vi "Define Test Suite (SimpleText Report).vi"(4 "timeout":i32=2000, 5 "register caller level (0)":i32, 6 "Verbose (F)":bool, 8 "error in (no error)":errorcluster, 9 "Report Path":path, 10 "Interactive":bool, 11 "Label (VI Title)":string) -> (0 "error out":errorcluster, 2 "Properties.Suite":refnum<class "Properties.Suite.lvclass">, 3 "Test Suite":refnum<class "Test Suite.lvclass">)   [LabVIEW 2020, in "Caraya.lvlib" / "Test Suite.lvclass"]
doc: "Registers the calling VI as a test suite. If Interactive is True, the interactive user interface is opened when the test suite is executed. If the Report Path is set, a report file will be generated with the test results.\n\n--\nCopyright © 2015 JKI All rights reserved.\n\nAuthor: Tomi Maila <tomi.maila@jki.net>\n\nThis library is provided \"AS IS\" ,WITHOUT WARRANTIES OR\nCONDITIONS OF ANY KIND, either express or implied.\n\nJKI -- jki.net"
uses:
  Test Suite.lvclass
  Properties.Suite/Properties.Suite.lvclass
  C:/projects/caraya/src/classes/Properties/Properties.lvclass
  Test Assert Factory/Test Assert Factory.lvclass
  Test Report.Default/Test Report.Default.lvclass
  C:/projects/caraya/src/classes/Test Report/Test Report.lvclass
  Test Suite.lvclass/Test Suite.ctl
  Properties.Suite/Properties.Suite.lvclass/Properties.Suite.ctl
  Caraya.lvlib
  Assert Factory Manager/Assert Factory Manager.lvclass
  Basic Test Manager/Basic Test Manager.lvclass
  Properties/Properties.lvclass
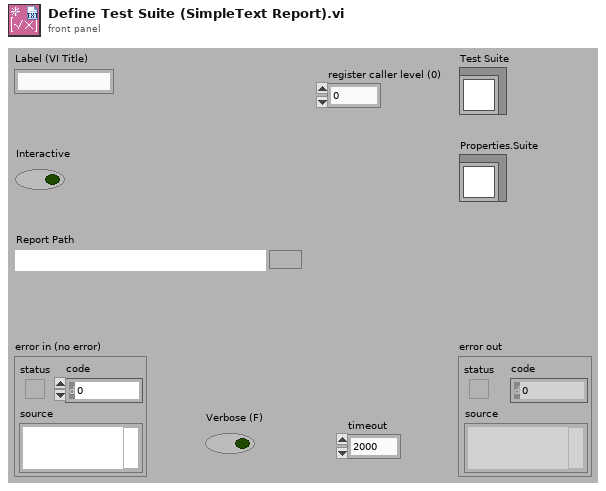
[diagram p1: front panel]
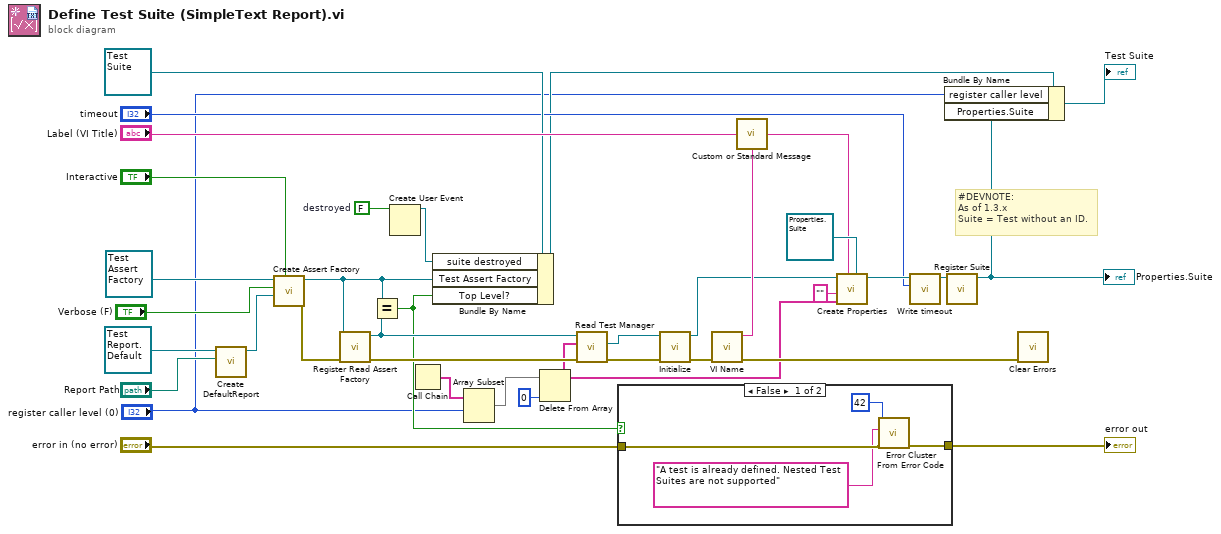
[diagram p0: block diagram]
diagram:
  w16 = FALSE  # destroyed
  # "#DEVNOTE:\nAs of 1.3.x\nSuite = Test without an ID."
  n1 = call "Create DefaultReport.vi"("Report Path"="Report Path", "Test Report.Default in"=refnum<class "Test Report.Default.lvclass"> refnum) -> ("Test Report.Default out"=w20:refnum<class "Test Report.Default.lvclass">)  [unwired: 8 in, 1 out]
  n2 = call "Create Assert Factory.vi"("Interactive"="Interactive", "Test Report"=w20, "Verbose (F)"="Verbose (F)", "Test Assert Factory in"=refnum<class "Test Assert Factory.lvclass"> refnum ("Caraya.lvlib:Test Assert Factory.lvclass")) -> ("error out"=w18:errorcluster, "Test Assert Factory out"=w19:refnum<class "Test Assert Factory.lvclass">)  [unwired: 6 in]
  n3 = call "Register Read Assert Factory.vi"("error in (no error)"=w18, "Test Assert Factory"=w19) -> ("error out"=w36:errorcluster, "Test Assert Factory"=w30:refnum<class "Test Assert Factory.lvclass">)  [unwired: 8 in]
  n4 = Equal?(x=w19, y=w30) -> (x = y?=w17:bool)
  n5 = Create User Event(user event datatype=w16) -> (user event=w15:refnum<user-event>)  [unwired: 1 in, 1 out]
  n6 = Call Chain() -> (call chain=w3:string[])
  n7 = Bundle By Name(cluster=refnum<class "Test Suite.lvclass"> refnum ("Test Suite"), "suite destroyed"=w15, "Test Assert Factory"=w19, "Top Level?"=w17) -> (w5:refnum<class "Test Suite.lvclass">)
  n8 = Array Subset(array=w3, index="register caller level (0)") -> (w2:string[])  [unwired: 1 in]
  n9 = Delete From Array(array=w2, index=0) -> (array with subset deleted=w11:string[])  [unwired: 1 in, 1 out]
  n10 = call-dynamic "Read Test Manager.vi"("error in (no error)"=w36, "VI Call Chain"=w11, "Assert Factory in"=w30) -> ("error out"=w34:errorcluster, "Basic Test Manager"=w27:refnum<class "Basic Test Manager.lvclass">)  [unwired: 6 in, 1 out]
  n11 = case shown="False" w17 {
    tunnel: [w41 w42] -> w29
    tunnel: "error in (no error)" -> [w40 w42]
    frame False {
      n12 = call <vilib>:"Error Cluster From Error Code.vi"("error in (no error)"=w40, "error message (\"\")"="A test is already defined. Nested Test Suites are not supported" ("error message (\"\")"), "error code (0)"=42) -> ("error out"=w41:errorcluster)  [unwired: 6 in]
    }
    frame True {
    }
  }
  "error out" <- w29
  n13 = call "Initialize.vi"("error in (no error)"=w34, "Test Manager in"=w27) -> ("error out"=w33:errorcluster, "Test Manager out"=w10:refnum<class "Basic Test Manager.lvclass">)  [unwired: 8 in]
  n14 = call "VI Name.vi"("error in (no error)"=w33) -> ("error out"=w32:errorcluster, "VI Name"=w35:string)  [unwired: 9 in]
  n15 = call "Custom or Standard Message.vi"("Custom Message"="Label (VI Title)", "Standard Message"=w35) -> ("Message"=w12:string)
  n16 = call "Create Properties.vi"("Properties in"=refnum<class "Properties.Suite.lvclass"> refnum ("Caraya.lvlib:Properties.Suite.lvclass"), "label"=w12, "call-chain"=w11, "self-id"="", "Test Manager"=w10) -> ("Properties out"=w9:refnum<class "Properties.Suite.lvclass">)  [unwired: 6 in]
  n17 = call "Write timeout.vi"("timeout"="timeout", "Properties.Suite in"=w9) -> ("Properties.Suite out"=w8:refnum<class "Properties.Suite.lvclass">)  [unwired: 9 in]
  n18 = call "Register Suite.vi"("Properties.Suite in"=w8) -> ("Properties.Suite out"=w6:refnum<class "Properties.Suite.lvclass">)  [unwired: 10 in]
  "Properties.Suite" <- w6
  n19 = Bundle By Name(cluster=w5, "register caller level"="register caller level (0)", "Properties.Suite"=w6) -> (→"Test Suite":refnum<class "Test Suite.lvclass">)
  n20 = call <vilib>:"Clear Errors.vi"("error in (no error)"=w32) -> ()  [unwired: 5 in, 2 out]
